vi "Handle Value Change.vi"(5 "VolatusAPI":refnum<class "VolatusAPI.lvclass">, 7 "CtlRef":refnum<vi>, 8 "error in (no error)":errorcluster, 9 "NewVal":variant, 10 "OldVal":variant, 11 "LoggingControl in":refnum<class "GroupLoggingControl.lvclass">) -> (0 "error out":errorcluster, 3 "LoggingControl out":refnum<class "GroupLoggingControl.lvclass">)   [LabVIEW 2020, in "VolatusGUIElements.lvlib" / "GroupLoggingControl.lvclass"]
uses:
  GroupLoggingControl.lvclass
  Volatus/VolatusAPI/VolatusAPI.lvclass
  GroupLoggingControl.lvclass/GroupLoggingControl.ctl
  Log Prompt Async.vi
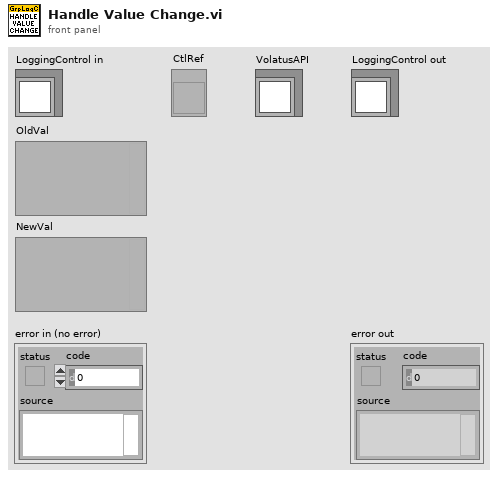
[diagram p1: front panel]
types:
  T1 = cluster{"Series":string, "Timestamp":string, "Targets":cluster{"Node":string, "Node Color":u32, "Groups":cluster{"Group":string, "Group Color":u32, "Button":bool}[]}[], "Groups":cluster{"Group":string, "Group Color":u32, "Button":bool}[]}
  T2 = typedef "VolatusGUIElements.lvlib/GroupLoggingControl.lvclass/Log Group.ctl" = cluster{"Status":T3, "Command Info":T4, "State":refnum<class "StringChannel.lvclass">, "Logging":bool}
  T3 = typedef "VolatusGUIElements.lvlib/GroupLoggingControl.lvclass/Log Group Status.ctl" = cluster{"Group":string, "Group Color":u32, "Button":bool}
  T4 = typedef "VolatusGUIElements.lvlib/GroupLoggingControl.lvclass/Command Info.ctl" = cluster{"Commanding":bool, "Cmd Time":dbl, "Group ID":string}
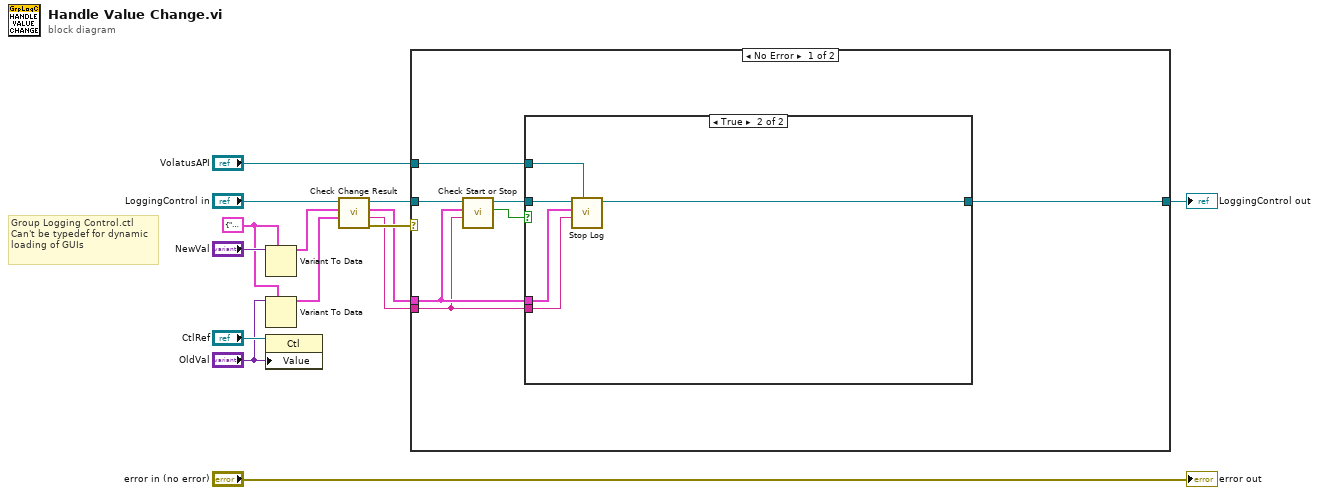
[diagram p0: block diagram]
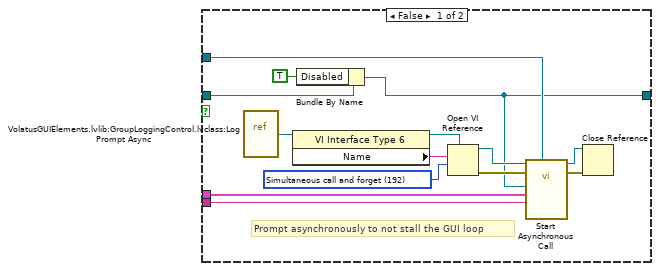
[diagram p2: hidden frame]
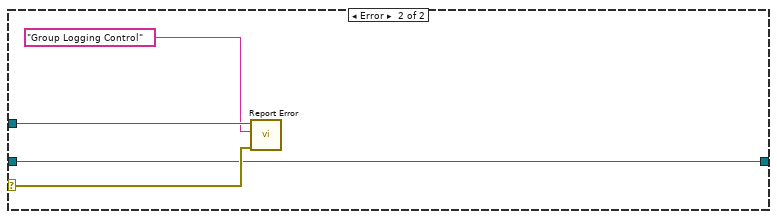
[diagram p3: hidden frame]
diagram:
  w1 = T1 {"Series"="", "Timestamp"="", "Targets"=[], "Groups"=[]} ("Group Logging Control")
  # "Group Logging Control.ctl Can't be typedef for dynamic loading of GUIs"
  n1 = Variant To Data(type=w1, Variant="NewVal") -> (data=w9:T1)  [unwired: 1 in, 1 out]
  n2 = Variant To Data(type=w1, Variant="OldVal") -> (data=w6:T1)  [unwired: 1 in, 1 out]
  n3 = property class="Ctl"(reference="CtlRef", "Value"="OldVal") -> ()  [unwired: 1 in, 2 out]
  n4 = call "Check Change Result.vi"("Old Val"=w6, "New Val"=w9, "GroupLoggingControl in"="LoggingControl in") -> ("error out"=w14:errorcluster, "Node (Empty = All)"=w2:string, "Log Group"=w3:T2, "GroupLoggingControl out"=w7:refnum<class "GroupLoggingControl.lvclass">)  [unwired: 5 in]
  n5 = case shown="No Error" w14 {
    selector: w14 -> [_ w44]
    tunnel: "VolatusAPI" -> [w21 w42]
    tunnel: w7 -> [w20 w43]
    tunnel: [w19 w43] -> w11
    tunnel: w3 -> [w17 _]
    tunnel: w2 -> [w16 _]
    frame No Error {
      n6 = call "Check Start or Stop.vi"("Target (All)"=w16, "Log Group (All)"=w17, "GroupLoggingControl in"=w20) -> ("Logging"=w15:bool, "GroupLoggingControl out"=w18:refnum<class "GroupLoggingControl.lvclass">)  [unwired: 6 in, 1 out]
      n7 = case shown="True" w15 {
        tunnel: w21 -> [w27 w39]
        tunnel: [w26 w38] -> w19
        tunnel: w18 -> [w24 w40]
        tunnel: w17 -> [w23 w37]
        tunnel: w16 -> [w22 w36]
        frame False {
          w30 = 192 items=["Record modifications"=1, "Open templates for editing"=2, "Prompt user to save"=4, "Prepare for reentrant run"=8, "Prompt to find missing subVIs"=16, "Hide loading dialog box"=32, "Enable simultaneous calls"=64, "Prepare to call and forget"=128, "Simultaneous call and forget"=192, "Prepare to call and collect"=256, "Simultaneous call and collect"=320]
          # "Prompt asynchronously to not stall the GUI loop"
          n8 = vi-ref "VolatusGUIElements.lvlib:GroupLoggingControl.lvclass:Log Prompt Async.vi"() -> (w28:refnum<vi>)
          n9 = property class="VI Interface Type 6"(reference=w28) -> (reference out=w31:refnum<vi>, "Name"=w29:string)  [unwired: 1 in, 1 out]
          n10 = Bundle By Name(cluster=w24, "Disabled"=TRUE) -> (w26:refnum<class "GroupLoggingControl.lvclass">)
          n11 = Open VI Reference(type specifier VI Refnum (for type only)=w31, vi path=w29, options=w30) -> (vi reference=w33:refnum<vi>, error out=w32:errorcluster)  [unwired: 3 in]
          n12 = call-by-ref "Start Asynchronous Call"(reference=w33, error in=w32, "VolatusAPI"=w27, "Target (All)"=w22, "Log Group (All)"=w23, "LoggingControl in"=w26) -> (reference out=w35:refnum<vi>, error out=w34:errorcluster)  [unwired: 8 in]
          n13 = Close Reference(reference=w35, error in (no error)=w34) -> ()  [unwired: 1 out]
        }
        frame True {
          n14 = call "Stop Log.vi"("VolatusAPI in"=w39, "Target (All)"=w36, "Log Group (All)"=w37, "GroupLoggingControl in"=w40) -> ("GroupLoggingControl out"=w38:refnum<class "GroupLoggingControl.lvclass">)  [unwired: 6 in, 1 out]
        }
      }
    }
    frame Error {
      n15 = call "Report Error.vi"("error in (no error)"=w44, "Context"="Group Logging Control", "VolatusAPI in"=w42) -> ()  [unwired: 7 in, 2 out]
    }
  }
  "LoggingControl out" <- w11
  "error out" <- "error in (no error)"
